vi "Parse Change CO3000 Ant Pol.vi"(8 "error in (no error)":errorcluster caption="에러 입력(에러 없음)", 10 "JSON string":string, 11 "Instrument Manager 입력":refnum<class "Instrument Manager.lvclass">) -> (0 "error out":errorcluster caption="에러 출력", 1 "Mast Index":i32=1, 2 "Antenna Pol":enum16{"H", "V"}(ring), 3 "Instrument Manager 출력":refnum<class "Instrument Manager.lvclass">, 5 "Change CO3000 Ant Pol Param":T1)   [LabVIEW 2023, in "Instrument Manager.lvclass"]
uses:
  Instrument Manager.lvclass
  Param Definition/Change CO3000 Ant Pol Param.ctl
  Instrument Manager.lvclass/Instrument Manager.ctl
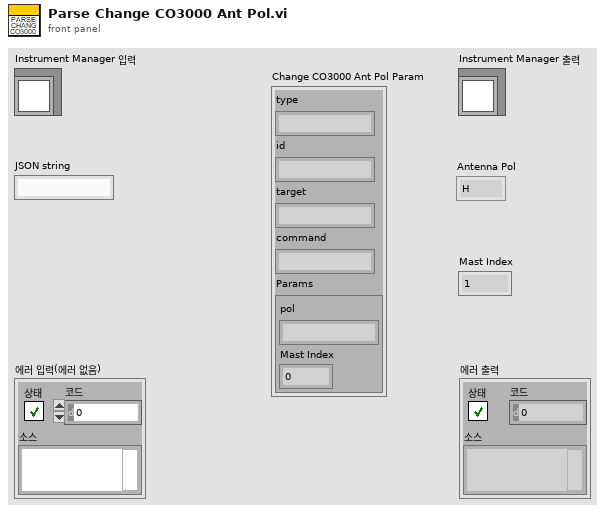
[diagram p1: front panel]
types:
  T1 = typedef "Instrument Manager.lvclass/Change CO3000 Ant Pol Param.ctl" = cluster{"type":string, "id":string, "target":string, "command":string, "Params":cluster{"pol":string, "Mast Index":i32}}
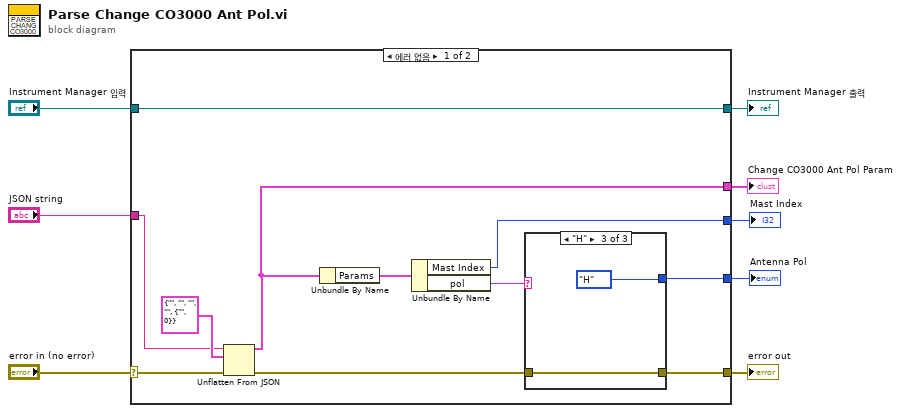
[diagram p0: block diagram]
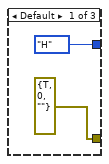
[diagram p2: hidden frame]
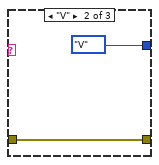
[diagram p3: hidden frame]
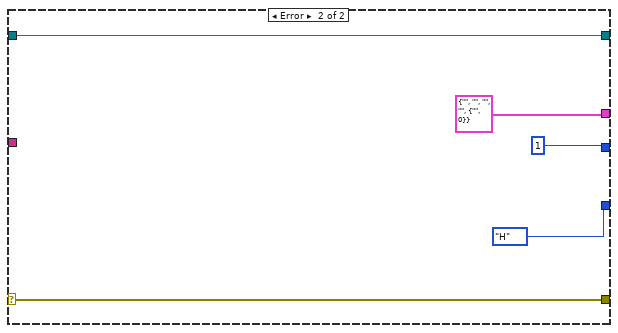
[diagram p4: hidden frame]
diagram:
  n1 = case shown="에러 없음" "error in (no error)" {
    selector: "error in (no error)" -> [w18 w30]
    tunnel: [w12 w30] -> w7
    tunnel: [w19 w29] -> w5
    tunnel: "Instrument Manager 입력" -> [w19 w29]
    tunnel: "JSON string" -> [w16 _]
    tunnel: [w11 enum16{"H", "V"}."H" ("Antenna Pol")] -> w3
    tunnel: [w10 T1 {"type"="", "id"="", "target"="", "command"="", "Params"={"pol"="", "Mast Index"=0}} ("Change CO3000 Ant Pol Param")] -> w2
    tunnel: [w9 1 ("Mast Index")] -> w1
    frame No Error {
      n2 = Unflatten From JSON(JSON string=w16, type and defaults=T1 {"type"="", "id"="", "target"="", "command"="", "Params"={"pol"="", "Mast Index"=0}} ("Change CO3000 Ant Pol Param"), error in (no error)=w18) -> (value=w10:T1, error out=w13:errorcluster)  [unwired: 4 in]
      n3 = Unbundle By Name(w10) -> ("Params"=w15:cluster{"pol":string, "Mast Index":i32})
      n4 = Unbundle By Name(w15) -> ("Mast Index"=w9:i32, "pol"=w14:string)
      n5 = case shown="\"H\"" w14 {
        tunnel: w13 -> [_ w23 w24]
        tunnel: [errorcluster {"status"=TRUE, "code"=0, "source"=""} ("error out") w23 w24] -> w12
        tunnel: [enum16{"H", "V"}."H" ("Antenna Pol") enum16{"H", "V"}."V" ("Antenna Pol") enum16{"H", "V"}."H" ("Antenna Pol")] -> w11
        frame Default {
        }
        frame "V" {
        }
        frame "H" {
        }
      }
    }
    frame Error {
    }
  }
  "error out" <- w7
  "Instrument Manager 출력" <- w5
  "Antenna Pol" <- w3
  "Change CO3000 Ant Pol Param" <- w2
  "Mast Index" <- w1
